vi "VI Tester About.vi"() -> ()   [LabVIEW 2017, in "GraphicalTestRunner.lvlib"]
uses:
  GraphicalTestRunner.lvlib
panel:
  out "Status":string
  out "Version":string
  in  "Website Button":bool
  in  "copyrights":bool
  in  "Cancel":bool
  # "VI Tester for LabVIEW"
  # "© 2007 - 2022 VI Tester Contributors. All Rights Reserved."
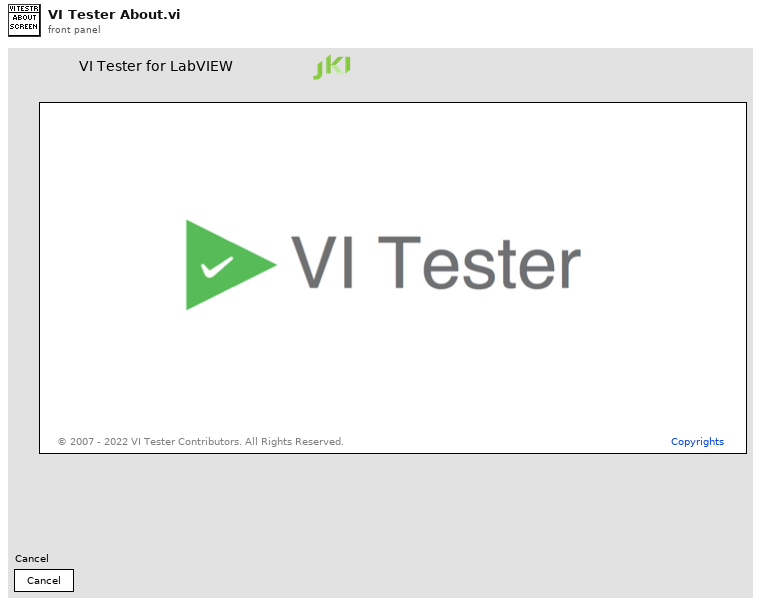
[diagram p1: front panel]
types:
  T1 = enum32{"Invalid", "Default", "Floating", "Floating/Auto-Hide", "Modal"}
  T2 = cluster{"Version":string, "Build Number":u32, "Build Date/Time":dbl}
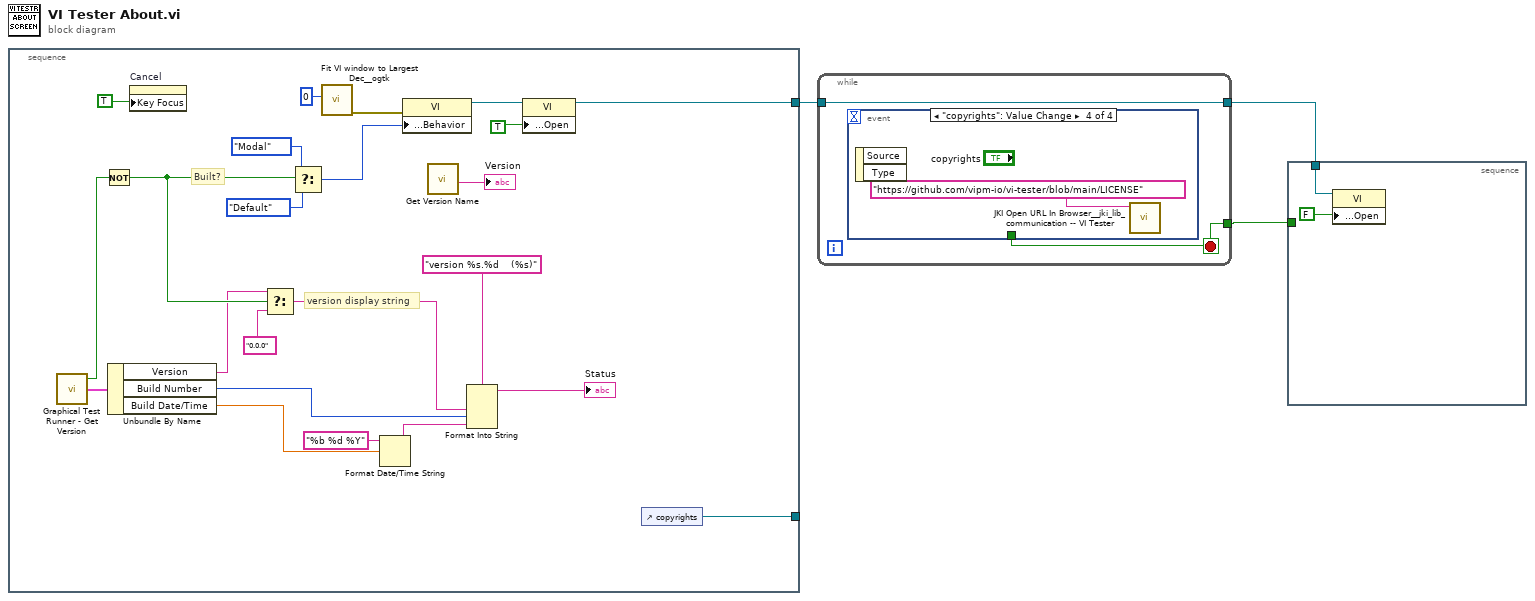
[diagram p0: block diagram]
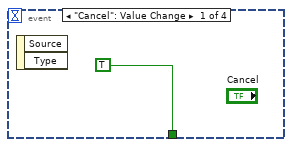
[diagram p2: hidden frame]
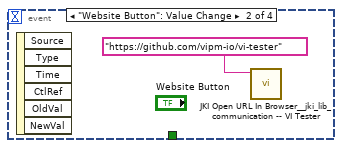
[diagram p3: hidden frame]
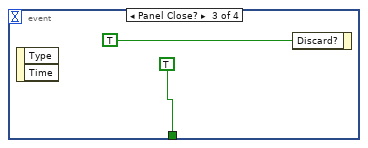
[diagram p4: hidden frame]
diagram:
  n1 = stacked-sequence {
    tunnel: [w6] -> w2
    tunnel: [w8] -> _
    frame #0 {
      # "Built?"
      # "version display string"
      n2 = call "Graphical Test Runner - Get Version.vi"() -> ("Version Info"=w24:T2, "Dev. Environment?"=w15:bool)  [unwired: 4 in]
      n3 = Not(x=w15) -> (.not. x?=w14:bool)
      n4 = Unbundle By Name(w24) -> ("Version"=w13:string, "Build Number"=w19:u32, "Build Date/Time"=w20:dbl)
      n5 = property on="Cancel" class="Bool"("Key Focus"=TRUE) -> ()  [unwired: 2 in, 2 out]
      n6 = Select(t=w13, s=w14, f="0.0.0") -> (s? t:f=w12:string)
      n7 = Select(t=T1."Modal" ("Front Panel Window:Behavior"), s=w14, f=T1."Default" ("Front Panel Window:Behavior")) -> (s? t:f=w16:T1)
      n8 = call <userlib>:"Fit VI window to Largest Dec__ogtk.vi"("border spacing (2 px)"=0) -> ("error out"=w10:errorcluster)  [unwired: 5 in, 1 out]
      n9 = Format Date/Time String(time format string (%c)="%b %d %Y", seconds (now)=w20) -> (date/time string=w21:string)  [unwired: 1 in]
      n10 = property class="VI"(error in=w10, "Front Panel Window:Behavior"=w16) -> (reference out=w7:refnum<vi>)  [unwired: 1 in, 1 out]
      n11 = call "Get Version Name.vi"() -> ("Version Name"=→"Version":string)
      n12 = Format Into String(format string="version %s.%d    (%s)", w12, w19, w21) -> (resulting string=→"Status":string)  [unwired: 2 in, 1 out]
      n13 = property class="VI"(reference=w7, "Front Panel.Open"=TRUE ("Front Panel Window:Open")) -> (reference out=w6:refnum<vi>)  [unwired: 1 in, 1 out]
      n14 = control-ref of="copyrights"() -> (w8:refnum<vi>)
    }
  }
  n15 = while {
    tunnel: [w28] -> w3
    tunnel: w2 -> [w27]
    tunnel: [w27] -> w1
    stop <- w28 stop-if-true
    n16 = event shown="[3] \"copyrights\": Value Change" {
      selector: _ -> [_ _ _ _]
      dyn-events: _ -> [_ _ _ _]
      timeout: _ -> [_ _ _ _]
      tunnel: [TRUE _ TRUE _] -> w28
      event "Cancel": Value Change {
        n17 = event-data() -> ()  [unwired: 1 in, 2 out]
      }
      event "Website Button": Value Change {
        n18 = event-data() -> ()  [unwired: 1 in, 6 out]
        n19 = call "JKI Open URL In Browser__jki_lib_communication -- VI Tester.vi"("url"="https://github.com/vipm-io/vi-tester") -> ()  [unwired: 5 in, 2 out]
      }
      event Panel Close? {
        n20 = event-data() -> ()  [unwired: 1 in, 2 out]
        n21 = event-data("Discard?"=TRUE) -> ()  [unwired: 1 in, 1 out]
      }
      event "copyrights": Value Change {
        n22 = event-data() -> ()  [unwired: 1 in, 2 out]
        n23 = call "JKI Open URL In Browser__jki_lib_communication -- VI Tester.vi"("url"="https://github.com/vipm-io/vi-tester/blob/main/LICENSE") -> ()  [unwired: 5 in, 2 out]
      }
    }
  }
  n24 = stacked-sequence {
    tunnel: w3 -> [_]
    tunnel: w1 -> [w34]
    frame #0 {
      n25 = property class="VI"(reference=w34, "Front Panel.Open"=FALSE ("Front Panel Window:Open")) -> ()  [unwired: 1 in, 2 out]
    }
  }
